vi "strings to line.vi"(11 "strings":string[](array[string])) -> (3 "line":T1)   [LabVIEW 2013, in "EIP Tags editor node.lvclass"]
uses:
  EIP Tags editor node.lvclass
  table line.ctl
  channel/EIP Tags Channel.lvclass
  <vilib>/NI/Tag Bus Module Framework/channel/channel classification.ctl
  configuration/eip tag types.ctl
  <vilib>/NI/Tag Bus Module Framework/channel/TBM channel.lvclass
  configuration/EIP Tags Configuration.lvclass
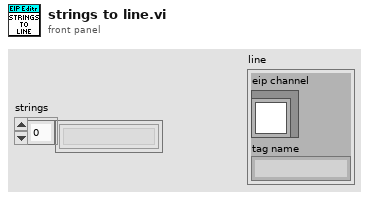
[diagram p1: front panel]
types:
  T1 = typedef "EIP Tags editor node.lvclass/table line.ctl" = cluster{"eip channel":refnum<class "EIP Tags Channel.lvclass">, "tag name":string}
  T2 = typedef "EIP Tags Configuration.lvclass/eip tag types.ctl" = enum16{"SINT", "INT", "DINT", "REAL", "BOOL", "STRING"}
  T3 = typedef "TBM channel.lvclass/channel classification.ctl" = enum16{"input data", "output data", "processing parameter", "processing result"}
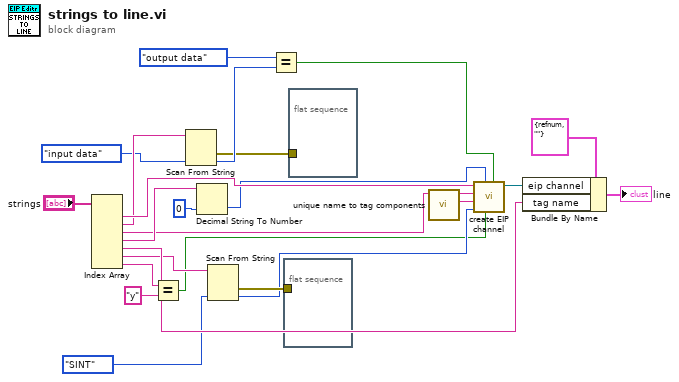
[diagram p0: block diagram]
diagram:
  n1 = Index Array(array="strings") -> (element #1=w21:string, element #2=w16:string, element #3=w8:string, element #4=w18:string, element #5=w22:string, element #6=w4:string, element #7=w3:string)  [unwired: 7 in]
  n2 = Equal?(x=w3, y="y") -> (x = y?=w1:bool)
  n3 = Scan From String(input string=w16, default 1=channel_classification."input data" ("channel classification")) -> (error out=w11:errorcluster, output 1=w14:T3)  [unwired: 3 in, 2 out]
  n4 = Decimal String To Number(string=w18, default (0L)=u32 0 ("default (0 I32)")) -> (number=w17:u32)  [unwired: 1 in, 1 out]
  n5 = Scan From String(input string=w4, default 1=eip_tag_types."SINT" ("eip tag type")) -> (error out=w7:errorcluster, output 1=w6:T2)  [unwired: 3 in, 2 out]
  n6 = Equal?(x=channel_classification."output data", y=w14) -> (x = y?=w12:bool)
  n7 = flat-sequence {
    tunnel: w7 -> [_]
    frame #0 {
    }
  }
  n8 = flat-sequence {
    tunnel: w11 -> [_]
    frame #0 {
    }
  }
  n9 = call "unique name to tag components.vi"("unique name"=w8) -> ("Tag Name"=w9:string, "Network Path"=w10:string)  [unwired: 9 in]
  n10 = call "create EIP channel.vi"("output?"=w12, "array?"=w1, "element index"=w17, "eip tag type"=w6, "Tag Name"=w9, "Network Path"=w10, "name"=w21) -> ("EthernetIP Channel out"=w20:refnum<class "EIP Tags Channel.lvclass">)  [unwired: 4 in]
  n11 = Bundle By Name(cluster=T1 {"eip channel"=refnum, "tag name"=""} ("line"), "eip channel"=w20, "tag name"=w22) -> (→"line":T1)
